vi "Move_Pole.vi"(0 "State":T1={"Tick"=0, "Phase"=0, "PhaseTicks"=0, "Level"=1, "Room"=0, "X10"=0, "Y10"=0, "VY10"=0, "Mode"=0, "Facing"=0, "Run"=0, "Vert"=0, "StandY"=0, "EntryX10"=0, "EntryY10"=0, "EntryMode"=0, "Lives"=4, "Score"=0, "NextLife"=10000, "KeyR"=0, "KeyB"=0, "KeyY"=0, "Torch"=FALSE, "FloorPhase"=0, "Dead"=FALSE, "LevelStart"=FALSE, "Quit"=FALSE, "Sound"=0, "Seed"=12345, "DemoStep"=0, "Tiles"=[], "World"=[], "Enemies"=[], "Highscores"=[], "Name"=[0, 0, 0], "Cursor"=0}, 7 "XA10":i32, 11 "error in":errorcluster) -> (4 "Mode":i32, 8 "Y10":i32, 15 "error out":errorcluster)   [LabVIEW 2020, in "GH_Engine.lvlib"]
doc: "Claude on a pole, one tick: slide down until a floor, fall off the lower end. Inline subVI of Player_Move."
uses:
  GH_Engine.lvlib
  Level/GH_Level.lvlib
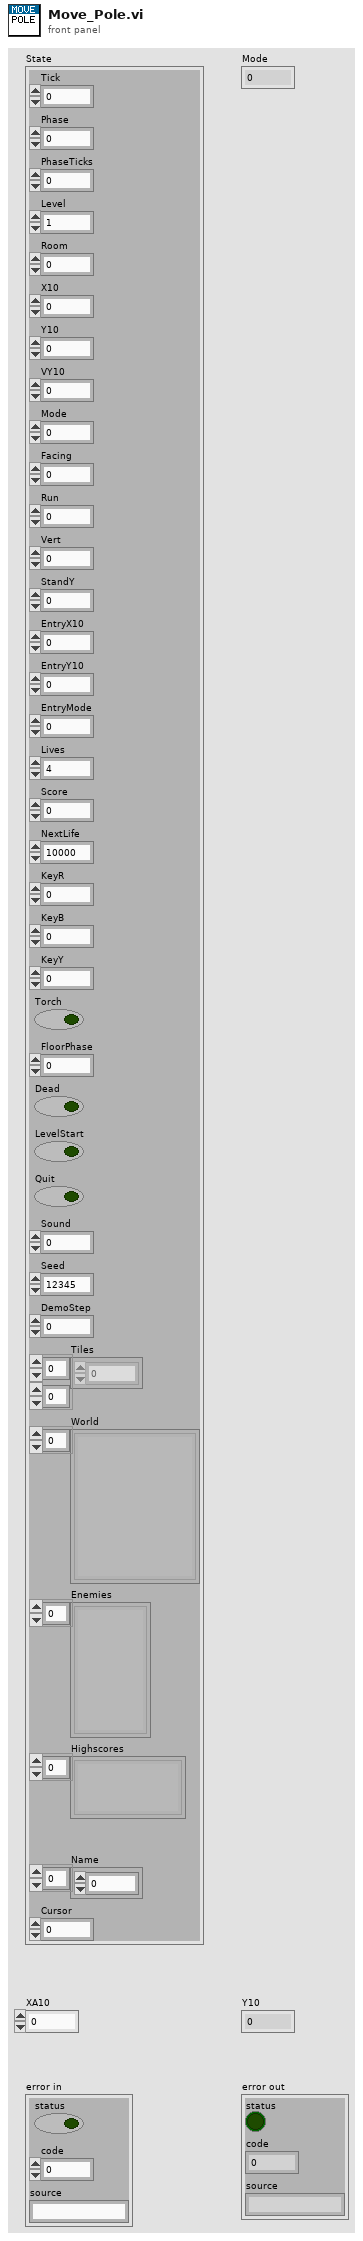
[diagram p1: front panel]
types:
  T1 = cluster{"Tick":u32, "Phase":i32, "PhaseTicks":i32, "Level":i32, "Room":i32, "X10":i32, "Y10":i32, "VY10":i32, "Mode":i32, "Facing":i32, "Run":i32, "Vert":i32, "StandY":i32, "EntryX10":i32, "EntryY10":i32, "EntryMode":i32, "Lives":i32, "Score":i32, "NextLife":i32, "KeyR":i32, "KeyB":i32, "KeyY":i32, "Torch":bool, "FloorPhase":i32, "Dead":bool, "LevelStart":bool, "Quit":bool, "Sound":i32, "Seed":u32, "DemoStep":i32, "Tiles":u8[][], "World":cluster{"ID":string, "Depth":i32, "Column":i32, "Tiles":u8[][]}[], "Enemies":cluster{"Kind":i32, "X10":i32, "Y10":i32, "Dir":i32, "Mode":i32}[], "Highscores":cluster{"Score":i32, "Name":string}[], "Name":i32[], "Cursor":i32}
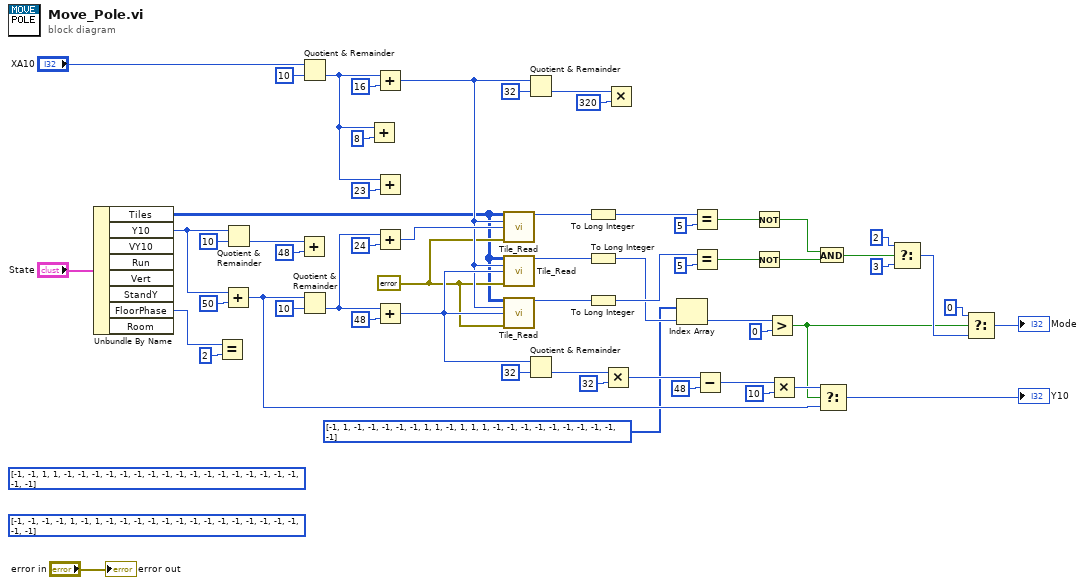
[diagram p0: block diagram]
diagram:
  w9 = errorcluster {"status"=FALSE, "code"=0, "source"=""} ("no error")
  (unwired) i32[] [-1, -1, -1, -1, 1, -1, 1, -1, -1, -1, -1, -1, -1, -1, -1, -1, -1, -1, -1, -1, -1, -1, -1] ("Ladder or rope")
  (unwired) i32[] [-1, -1, 1, 1, -1, -1, -1, -1, -1, -1, -1, -1, -1, -1, -1, -1, -1, -1, -1, -1, -1, -1, -1] ("Thin floor")
  n1 = Unbundle By Name("State") -> ("Tiles"=w4:u8[][], "Y10"=w5:i32, "FloorPhase"=w6:i32)  [unwired: 5 out]
  n2 = Equal?(x=w6, y=2) -> ()  [unwired: 1 out]
  n3 = Add(x=w5, y=50) -> (x+y=w23:i32)
  n4 = Quotient & Remainder(x=w5, y=10) -> (floor(x/y)=w17:i32)  [unwired: 1 out]
  n5 = Add(x=w17, y=48) -> ()  [unwired: 1 out]
  n6 = Quotient & Remainder(x="XA10", y=10) -> (floor(x/y)=w11:i32)  [unwired: 1 out]
  n7 = Quotient & Remainder(x=w23, y=10) -> (floor(x/y)=w25:i32)  [unwired: 1 out]
  n8 = Add(x=w11, y=8) -> ()  [unwired: 1 out]
  n9 = Add(x=w11, y=16) -> (x+y=w13:i32)
  n10 = Add(x=w11, y=23) -> ()  [unwired: 1 out]
  n11 = Add(x=w25, y=24) -> (x+y=w34:i32)
  n12 = Add(x=w25, y=48) -> (x+y=w27:i32)
  n13 = call "Tile_Read.vi"("Tiles"=w4, "X"=w13, "Y"=w34, "error in"=w9) -> ("Tile"=w35:u8)  [unwired: 10 in, 1 out]
  n14 = call "Tile_Read.vi"("Tiles"=w4, "X"=w13, "Y"=w27, "error in"=w9) -> ("Tile"=w28:u8)  [unwired: 10 in, 1 out]
  n15 = call "Tile_Read.vi"("Tiles"=w4, "X"=w13, "Y"=w27, "error in"=w9) -> ("Tile"=w40:u8)  [unwired: 10 in, 1 out]
  n16 = Quotient & Remainder(x=w13, y=32) -> (floor(x/y)=w20:i32)  [unwired: 1 out]
  n17 = Quotient & Remainder(x=w27, y=32) -> (floor(x/y)=w52:i32)  [unwired: 1 out]
  n18 = To Long Integer(number=w35) -> (32bit integer=w36:i32)
  n19 = To Long Integer(number=w28) -> (32bit integer=w29:i32)
  n20 = To Long Integer(number=w40) -> (32bit integer=w41:i32)
  n21 = Multiply(x=w52, y=32) -> (x*y=w54:i32)
  n22 = Multiply(x=w20, y=320) -> ()  [unwired: 1 out]
  n23 = Index Array(array=i32[] [-1, 1, -1, -1, -1, -1, -1, 1, 1, -1, 1, 1, 1, -1, -1, -1, -1, -1, -1, -1, -1, -1, -1] ("Solid"), index=w29) -> (element=w30:i32)
  n24 = Equal?(x=w36, y=5) -> (x = y?=w38:bool)
  n25 = Equal?(x=w41, y=5) -> (x = y?=w43:bool)
  n26 = Subtract(x=w54, y=48) -> (x-y=w56:i32)
  n27 = Not(x=w38) -> (.not. x?=w39:bool)
  n28 = Not(x=w43) -> (.not. x?=w44:bool)
  n29 = Greater?(x=w30, y=0) -> (0:w32:bool)
  n30 = Multiply(x=w56, y=10) -> (x*y=w58:i32)
  n31 = And(x=w39, y=w44) -> (x .and. y?=w45:bool)
  n32 = Select(t=w58, s=w32, f=w23) -> (s? t:f=→"Y10":i32)
  n33 = Select(t=2, s=w45, f=3) -> (s? t:f=w49:i32)
  n34 = Select(t=0, s=w32, f=w49) -> (s? t:f=→"Mode":i32)
  "error out" <- "error in"
